vi "Find Interface.vi"(8 "error in (no error)":errorcluster, 10 "Interface Name":string, 11 "Object Type in":refnum<k24>) -> (0 "error out":errorcluster, 2 "Interface Type":refnum<k24>, 3 "Object Type out":refnum<k24>)   [LabVIEW 2026, in "ToastNotification.lvlib" / "Reflection DotNet.lvlib"]
doc: "Native System.Type.GetInterface call. Borrow Object Type in and acquire Interface Type for Interface Name. A null interface result means the interface is not implemented. Object Type out is an input alias. Caller closes the acquired interface Type, not the borrowed object Type."
uses:
  Reflection DotNet.lvlib
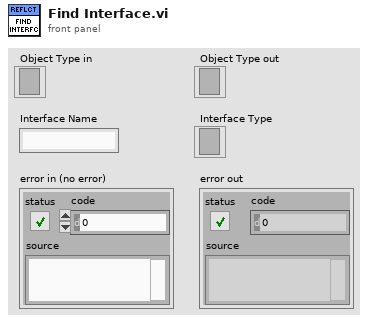
[diagram p1: front panel]
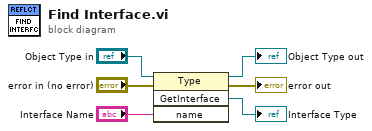
[diagram p0: block diagram]
diagram:
  n1 = invoke class="Type" method="GetInterface"(reference="Object Type in", error in="error in (no error)", "name"="Interface Name") -> (reference out=→"Object Type out":refnum<k24>, error out=→"error out":errorcluster, "GetInterface"=→"Interface Type":refnum<k24>)  [unwired: 1 in, 1 out]
